vi "session.vi"() -> ()   [LabVIEW 2026]
uses:
  <vilib>/REV Custom Controls/REVSparkRefnum.ctl
  <resource>/objmgr/REVSpark.rc
panel:
  in  "User Defined Refnum Tag":refnum<k21>
  in  "User Defined Refnum":refnum<k20>
  out "Array":cluster{"string":string, bool, bool, i16}[](array[cluster])
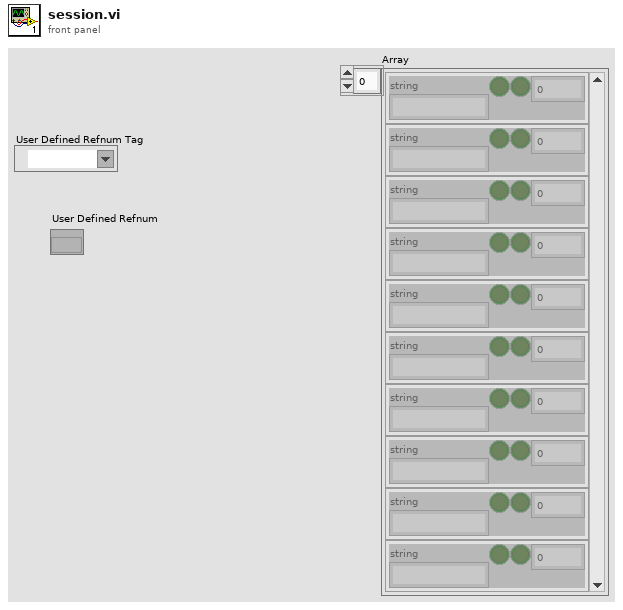
[diagram p1: front panel]
types:
  T1 = typedef "REVSparkRefnum.ctl" = refnum<k21>
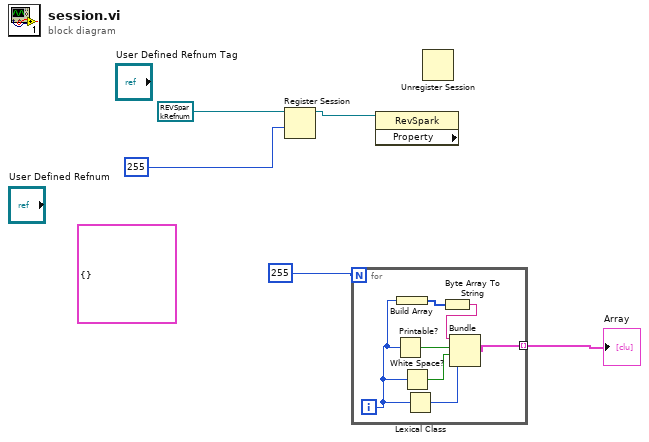
[diagram p0: block diagram]
diagram:
  (unwired) cluster{} {}
  n1 = Register Session(9:u64 255, 11:T1 refnum ("REV Spark Refnum")) -> (3:w1:T1)  [unwired: 3 in, 1 out]
  n2 = for {
    N: 255 -> [_]
    tunnel: [w10] -> w4 mode=indexing
    i -> [w7]
    n3 = Printable?(1:w7) -> (0:w9:bool)
    n4 = Build Array(w7) -> (w12:i32[])
    n5 = White Space?(1:w7) -> (0:w8:bool)
    n6 = Lexical Class(1:w7) -> (0:w6:i16)
    n7 = Byte Array To String(unsigned byte array=w12) -> (string=w11:string)
    n8 = Bundle("string"=w11, w9, w8, w6) -> (w10:cluster{"string":string, bool, bool, i16})  [unwired: 1 in]
  }
  "Array" <- w4
  n9 = property class="RevSpark" props=[](reference=w1) -> ()  [unwired: 1 in, 3 out]
  n10 = Unregister Session() -> ()  [unwired: 2 in, 1 out]
